vi "Prime Number.vi"() -> ()   [LabVIEW 2026]
panel:
  out "Result":string
  in  "Input Number":i32
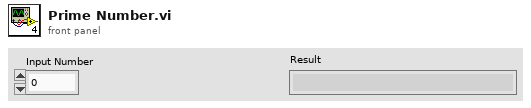
[diagram p1: front panel]
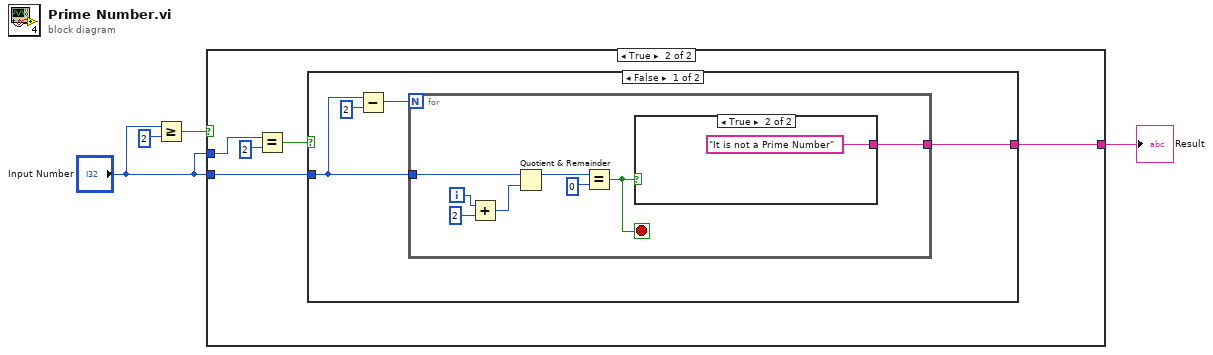
[diagram p0: block diagram]
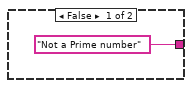
[diagram p2: hidden frame]
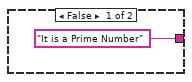
[diagram p3: hidden frame]
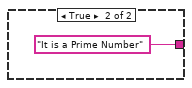
[diagram p4: hidden frame]
diagram:
  n1 = Greater Or Equal?(x="Input Number", y=2) -> (x >= y?=w3:bool)
  n2 = case shown="True" w3 {
    tunnel: "Input Number" -> [_ w10]
    tunnel: ["Not a Prime number" w9] -> w2
    tunnel: "Input Number" -> [_ w8]
    frame False {
    }
    frame True {
      n3 = Equal?(x=w8, y=2) -> (x = y?=w6:bool)
      n4 = case shown="False" w6 {
        tunnel: w10 -> [w12 _]
        tunnel: [w11 "It is a Prime Number"] -> w9
        frame False {
          n5 = Subtract(x=w12, y=2) -> (x-y=w13:i32)
          n6 = for {
            N: w13 -> [_]
            tunnel: w12 -> [w22]
            tunnel: [w16] -> w11
            i -> [w21]
            stop <- w15 stop-if-true
            n7 = Add(x=w21, y=2) -> (x+y=w19:i32)
            n8 = Quotient & Remainder(x=w22, y=w19) -> (x-y*floor(x/y)=w18:i32)  [unwired: 1 out]
            n9 = Equal?(x=w18, y=0) -> (x = y?=w15:bool)
            n10 = case shown="True" w15 {
              tunnel: ["It is a Prime Number" "It is not a Prime Number"] -> w16
              frame False {
              }
              frame True {
              }
            }
          }
        }
        frame True {
        }
      }
    }
  }
  "Result" <- w2
